vi "destroy.vi"(8 "error in (no error)":errorcluster, 11 "simple_html_chat_ui in":refnum<class "simple_html_chat_ui.lvclass">) -> (0 "error out":errorcluster, 3 "simple_html_chat_ui out":refnum<class "simple_html_chat_ui.lvclass">)   [LabVIEW 2020, in "simple_html_chat_ui.lvclass"]
uses:
  simple_html_chat_ui.lvclass
  simple_html_chat_ui.lvclass/simple_html_chat_ui.ctl
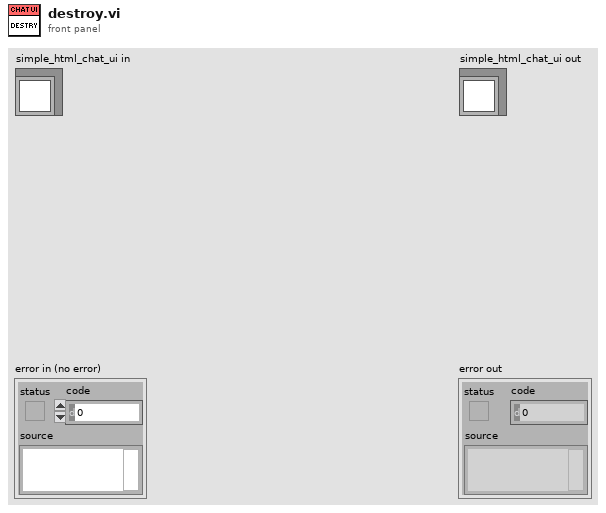
[diagram p1: front panel]
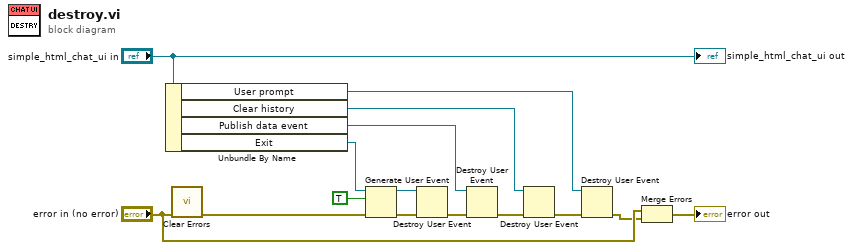
[diagram p0: block diagram]
diagram:
  n1 = Unbundle By Name("simple_html_chat_ui in") -> ("User prompt"=w1:refnum<user-event>, "Clear history"=w2:refnum<user-event>, "Publish data event"=w6:refnum<user-event>, "Exit"=w11:refnum<user-event>)
  n2 = call <vilib>:"Clear Errors.vi"("error in (no error)"="error in (no error)") -> ("error out"=w12:errorcluster)  [unwired: 5 in, 1 out]
  n3 = Generate User Event(user event=w11, event data cluster=TRUE ("event data"), error in=w12) -> (user event out=w8:refnum<user-event>, error out=w9:errorcluster)  [unwired: 1 in]
  n4 = Destroy User Event(user event=w8, error in=w9) -> (error out=w7:errorcluster)
  n5 = Destroy User Event(user event=w6, error in=w7) -> (error out=w5:errorcluster)
  n6 = Destroy User Event(user event=w2, error in=w5) -> (error out=w4:errorcluster)
  n7 = Destroy User Event(user event=w1, error in=w4) -> (error out=w3:errorcluster)
  n8 = Merge Errors("error in (no error)", w3) -> (→"error out":errorcluster)
  "simple_html_chat_ui out" <- "simple_html_chat_ui in"
